vi "Read Agent Public Key Data.vi"(8 "error in (no error)":errorcluster, 11 "agent public key":T2) -> (0 "error out":errorcluster, 2 "value":T1)   [LabVIEW 2017, in "libssh2.lvlib"]
doc: "Read the data of an agent public key."
uses:
  libssh2.lvlib
  Agent Public Key Refnum.ctl
  libssh2_agent_publickey.ctl
  Acquire Agent.vi
  Release Agent.vi
  Acquire Session.vi
  Release Session.vi
  Read Agent Public Key Refnum.vi
  Read Agent Refnum.vi
  Read Session Refnum.vi
  <vilib>/Utility/semaphor.llb/Acquire Semaphore.vi
  <vilib>/Utility/semaphor.llb/Release Semaphore.vi
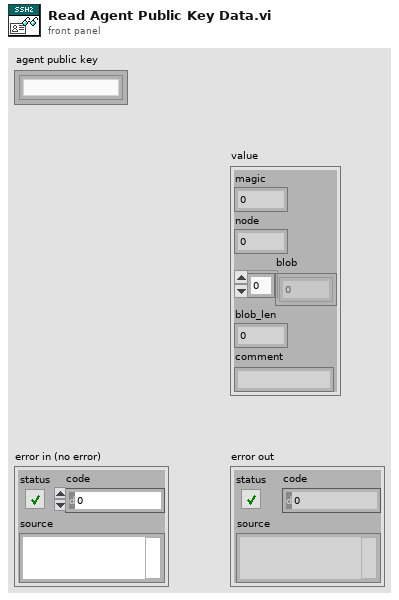
[diagram p1: front panel]
types:
  T1 = typedef "libssh2.lvlib/libssh2_agent_publickey.ctl" = cluster{"magic":u32, "node":u64, "blob":u8[], "blob_len":u64, "comment":string}
  T2 = typedef "libssh2.lvlib/Agent Public Key Refnum.ctl" = refnum<k1>
  T3 = cluster{"magic":u32, "node":u32, "blob":u32, "blob_len":u32, "comment":u32}
  T4 = cluster{"magic":u32, "padding<0>":u32, "node":u64, "blob":u64, "blob_len":u64, "comment":u64}
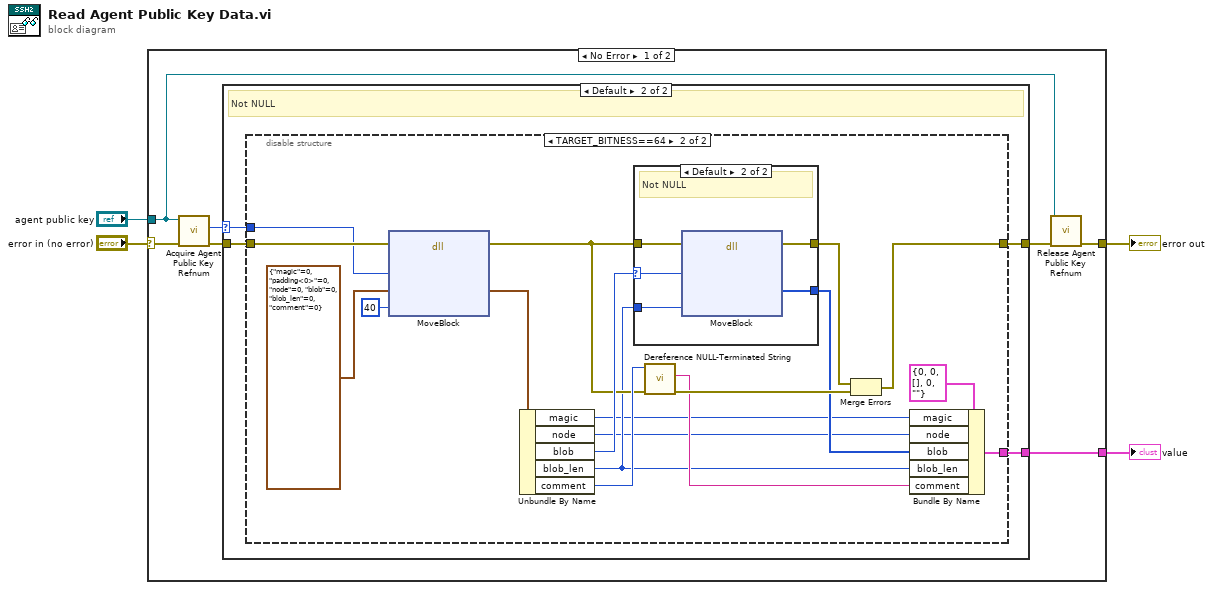
[diagram p0: block diagram]
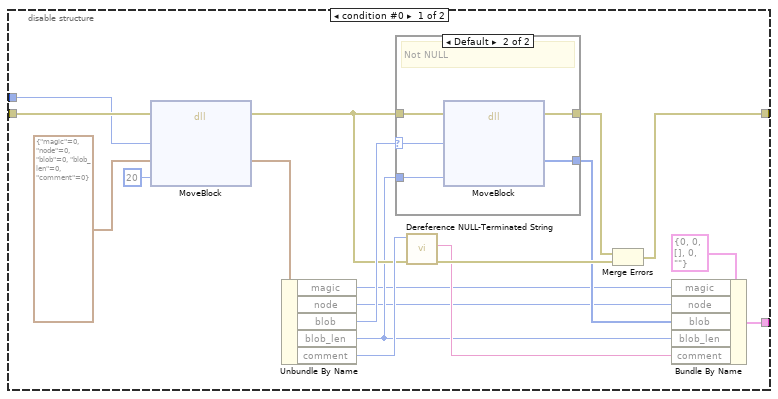
[diagram p3: hidden frame]
diagram:
  n1 = case shown="No Error" "error in (no error)" {
    selector: "error in (no error)" -> [w8 w63]
    tunnel: "agent public key" -> [w5 _]
    tunnel: [w6 w63] -> w3
    tunnel: [w7 _] -> w1
    frame No Error {
      n2 = call "Acquire Agent Public Key Refnum.vi"("error in (no error)"=w8, "agent public key"=w5) -> ("error out"=w11:errorcluster, "libssh2_agent_publickey*"=w9:u64)  [unwired: 8 in]
      n3 = case shown="Default" w9 {
        selector: w9 -> [_ w14]
        tunnel: w11 -> [w12 w16]
        tunnel: [w12 w15] -> w10
        tunnel: [_ w13] -> w7
        frame 0 {
          # "NULL"
        }
        frame Default {
          # "Not NULL"
          n4 = disable-structure shown="TARGET_BITNESS==64" {
            disable-tunnel: w16 -> [w34 w57]
            disable-tunnel: [w30 w53] -> w15
            disable-tunnel: w14 -> [w29 w52]
            disable-tunnel: [w21 w44] -> w13
            frame condition #0 {
              n5 = dll-call lib="LabVIEW" fn="MoveBlock"(error in=w34, "ps"=w29, "pd"=T3 {"magic"=0, "node"=0, "blob"=0, "blob_len"=0, "comment"=0}, "size"=u64 20) -> (error out=w26:errorcluster, "pd"=w24:T3)  [unwired: 5 in, 1 out]
              n6 = Unbundle By Name(w24) -> ("magic"=w17:u32, "node"=w18:u32, "blob"=w28:u32, "blob_len"=w19:u32, "comment"=w27:u32)
              n7 = case shown="Default" w28 {
                selector: w28 -> [_ w36]
                tunnel: w19 -> [_ w39]
                tunnel: [_ w38] -> w20
                tunnel: [_ w37] -> w31
                tunnel: w26 -> [_ w35]
                frame 0 {
                  # "NULL"
                }
                frame Default {
                  # "Not NULL"
                  n8 = dll-call lib="LabVIEW" fn="MoveBlock"(error in=w35, "ps"=w36, "size"=w39) -> (error out=w37:errorcluster, "pd"=w38:u8[])  [unwired: 6 in, 1 out]
                }
              }
              n9 = call "Dereference NULL-Terminated String.vi"("error in (no error)"=w26, "char*"=w27) -> ("error out"=w32:errorcluster, "string"=w22:string)  [unwired: 8 in]
              n10 = Merge Errors(w31, w32) -> (w30:errorcluster)
              n11 = Bundle By Name(cluster=T1 {"magic"=0, "node"=0, "blob"=[], "blob_len"=0, "comment"=""} ("libssh2_agent_publickey"), "magic"=w17, "node"=w18, "blob"=w20, "blob_len"=w19, "comment"=w22) -> (w21:T1)
            }
            frame condition #1 (active) {
              n12 = dll-call lib="LabVIEW" fn="MoveBlock"(error in=w57, "ps"=w52, "pd"=T4 {"magic"=0, "padding<0>"=0, "node"=0, "blob"=0, "blob_len"=0, "comment"=0}, "size"=u64 40) -> (error out=w49:errorcluster, "pd"=w47:T4)  [unwired: 5 in, 1 out]
              n13 = Unbundle By Name(w47) -> ("magic"=w40:u32, "node"=w41:u64, "blob"=w51:u64, "blob_len"=w42:u64, "comment"=w50:u64)
              n14 = case shown="Default" w51 {
                selector: w51 -> [_ w60]
                tunnel: w42 -> [_ w58]
                tunnel: [_ w62] -> w43
                tunnel: [_ w61] -> w54
                tunnel: w49 -> [_ w59]
                frame 0 {
                  # "NULL"
                }
                frame Default {
                  # "Not NULL"
                  n15 = dll-call lib="LabVIEW" fn="MoveBlock"(error in=w59, "ps"=w60, "size"=w58) -> (error out=w61:errorcluster, "pd"=w62:u8[])  [unwired: 6 in, 1 out]
                }
              }
              n16 = call "Dereference NULL-Terminated String.vi"("error in (no error)"=w49, "char*"=w50) -> ("error out"=w55:errorcluster, "string"=w45:string)  [unwired: 8 in]
              n17 = Merge Errors(w54, w55) -> (w53:errorcluster)
              n18 = Bundle By Name(cluster=T1 {"magic"=0, "node"=0, "blob"=[], "blob_len"=0, "comment"=""} ("libssh2_agent_publickey"), "magic"=w40, "node"=w41, "blob"=w43, "blob_len"=w42, "comment"=w45) -> (w44:T1)
            }
          }
        }
      }
      n19 = call "Release Agent Public Key Refnum.vi"("error in (no error)"=w10, "agent public key"=w5) -> ("error out"=w6:errorcluster)  [unwired: 9 in]
    }
    frame Error {
    }
  }
  "error out" <- w3
  "value" <- w1
